vi "NanonisGetSampleTime.vi"(8 "error in (no error)":errorcluster, 11 "String input":string="string test") -> (0 "error out":errorcluster, 3 "String output":string)   [LabVIEW 2011]
uses:
  <userlib>/Nanonis Prog Interface/Nanonis Prog Interface.lvlib
panel:
  out "Application ref out":refnum<vi>
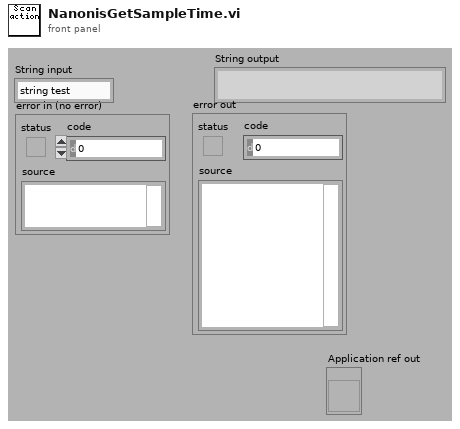
[diagram p1: front panel]
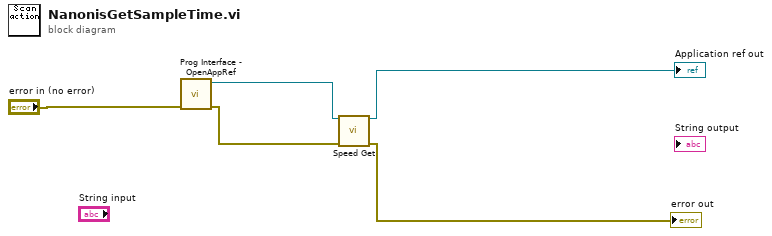
[diagram p0: block diagram]
diagram:
  n1 = call <userlib>:"Prog Interface - OpenAppRef.vi"("Error in (no error)"="error in (no error)") -> ("Error out"=w4:errorcluster, "Application reference"=w1:refnum<vi>)  [unwired: 5 in]
  n2 = call <userlib>:"Speed Get.vi"("Application ref in"=w1, "error in (no error)"=w4) -> ("Application ref out"=→"Application ref out":refnum<vi>, "error out"=→"error out":errorcluster)  [unwired: 9 in, 3 out]
